vi "Burst Clock (Host).vi"() -> ()   [LabVIEW 2021]
uses:
  <vilib>/userDefined/High Color/nirio_resource_hc.ctl
  5a54fa91-9ec7-467a-a88a-b72ee3603559.vi
  <vilib>/rvi/interface/RandomDataEmulation/nirviRandomDataOpen.vi
  <vilib>/rvi/interface/common/niFpgaCacheSessionInfoDynamic.vi
  <vilib>/FPGAPlugInAG/Dynamic/niLvFpga_Run_Dynamic.vi
  <vilib>/Utility/error.llb/Error Cluster From Error Code.vi
  <vilib>/rvi/errors/niLvFpgaAdjustHostInterfaceError.vi
  <vilib>/FPGAPlugInAG/Dynamic/niLvFpga_Close_Dynamic.vi
  <vilib>/rvi/interface/nirviOpenFPGA/nirviOpenFPGA.xnode
  Burst Clock (FPGA).vi
  <vilib>/rvi/interface/nirviMethod/nirviMethod.xnode
  <vilib>/rvi/interface/nirviReadWriteControl/nirviReadWriteControl.xnode
  <vilib>/rvi/interface/nirviCloseFPGA/nirviCloseFPGA.xnode
  <vilib>/rvi/interface/Simulation/niFpgaSimulationCallBeginRW.vi
  <vilib>/FPGAPlugInAG/Dynamic/niLvFpga_Reset_Dynamic.vi
  NiFpgaLv.dll
  <vilib>/FPGAPlugInAG/Dynamic/niLvFpga_WriteFifo_Dynamic.vi
  <vilib>/rvi/errors/niLvFpgaMergeErrorWithErrorCode.vi
panel:
  in  "Resource Name":T1 caption="RIO Device"
  in  "Stop":bool
  in  "Go":bool
  in  "Array":cluster{"Clocks":u16, "Idle":u16}[](array[cluster])=[{"Clocks"=5, "Idle"=3}]
  out "error out":errorcluster
  in  "error in (no error)":errorcluster
  # "To Simulate:\n1. Navigate to \"Project -> Properties -> Conditional Disable Signals\" and set \"FPGA_SIM\" to \"TRUE\".\n2. Right-click on the FPGA Target and set \"Select Execution Mode\" to \"Simulation (Simulated I/O)\" \n\nTo Run on FPGA:\n1. Navigate to \"Project -> Properties -> Conditional Disable Signals\" and set \"FPGA_SIM\" to \"FALSE\".\n2. Right-click on the FPGA Target and set \"Select Execution Mode\" to \"FPGA Target\""
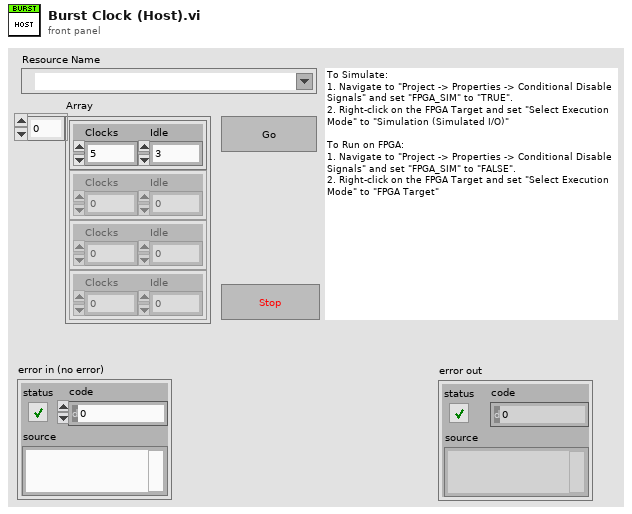
[diagram p1: front panel]
types:
  T1 = typedef "nirio_resource_hc.ctl" = tag
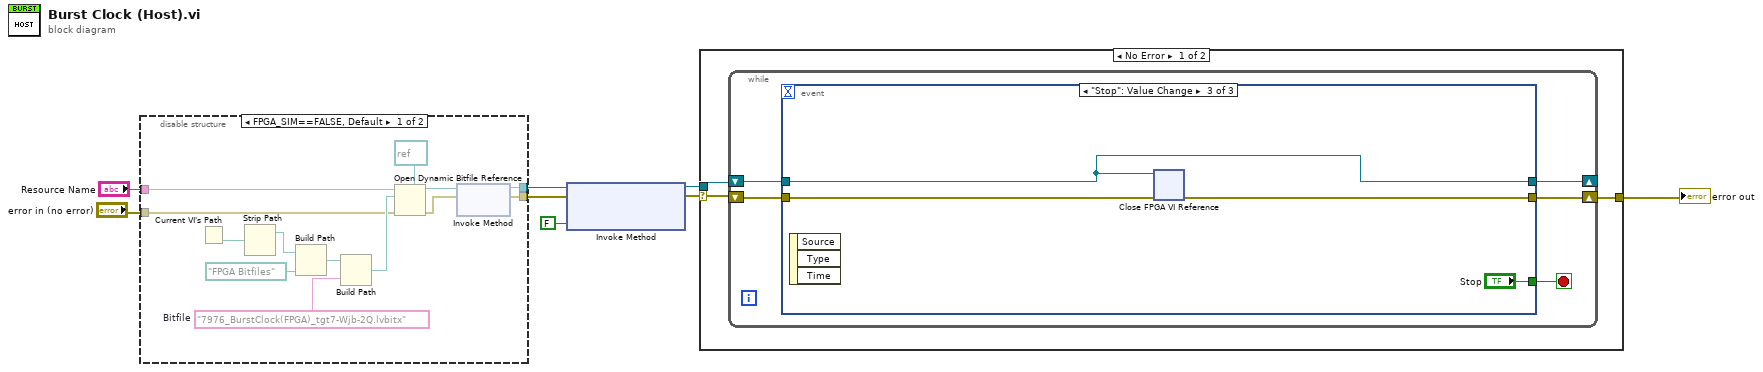
[diagram p0: block diagram]
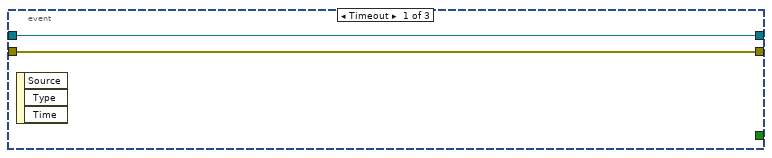
[diagram p2: hidden frame]
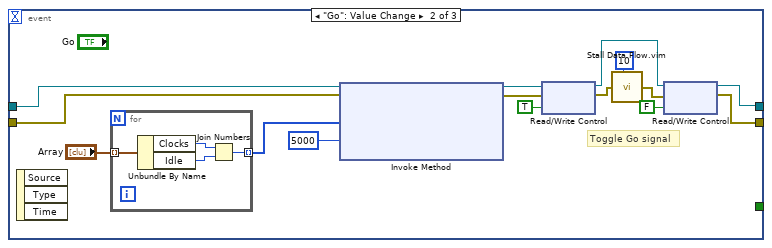
[diagram p3: hidden frame]
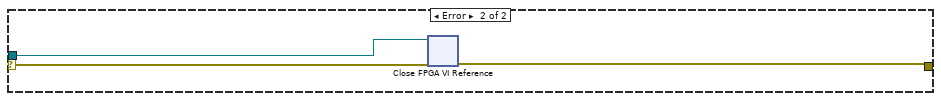
[diagram p4: hidden frame]
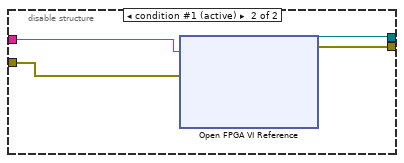
[diagram p5: hidden frame]
diagram:
  n1 = disable-structure shown="FPGA_SIM==FALSE, Default" {
    disable-tunnel: [w21 w23] -> w3
    disable-tunnel: [w20 w24] -> w4
    disable-tunnel: "error in (no error)" -> [w12 w25]
    disable-tunnel: "Resource Name" -> [w9 w22]
    frame condition #0 {
      w10 = "7976_BurstClock(FPGA)_tgt7-Wjb-2Q.lvbitx"  # Bitfile
      n2 = Current VI's Path() -> (path=w14:path)
      n3 = Strip Path(path=w14) -> (stripped path=w13:path)  [unwired: 1 out]
      n4 = Build Path(base path=w13, name or relative path=path "FPGA Bitfiles") -> (appended path=w18:path)
      n5 = Build Path(base path=w18, name or relative path=w10) -> (appended path=w19:path)
      n6 = Open Dynamic Bitfile Reference(0:w9, 1:w19, 3:w12, 4:refnum<k20> refnum ("FPGA Interface")) -> (5:w16:refnum<k20>, 8:w15:errorcluster)  [unwired: 1 in]
      n7 = xnode "Invoke Method"("FPGA VI Reference In"=w16, "error in"=w15) -> ("FPGA VI Reference Out"=w21:refnum<k20>, "error out"=w20:errorcluster)
    }
    frame condition #1 (active) {
      n8 = xnode "Open FPGA VI Reference"("error in"=w25, "resource name"=w22) -> ("FPGA VI Reference Out"=w23:refnum<k20>, "error out"=w24:errorcluster)
    }
  }
  n9 = xnode "Invoke Method"("FPGA VI Reference In"=w3, "error in"=w4, "Wait Until Done (F)"=FALSE) -> ("FPGA VI Reference Out"=w2:refnum<k20>, "error out"=w1:errorcluster)
  n10 = case shown="No Error" w1 {
    selector: w1 -> [w26 w61]
    tunnel: [w28 w59] -> w8
    tunnel: w2 -> [w27 w60]
    frame No Error {
      n11 = while {
        shift-right: [w30] -> w28
        shift-left: w26 -> [w33]
        shift-right: [w31] -> _
        shift-left: w27 -> [w32]
        stop <- w29 stop-if-true
        n12 = event shown="[2] \"Stop\": Value Change" {
          selector: _ -> [_ _ _]
          dyn-events: _ -> [_ _ _]
          timeout: _ -> [_ _ _]
          tunnel: w33 -> [w34 w50 w57]
          tunnel: w32 -> [w35 w49 w55]
          tunnel: [w35 w37 w55] -> w31
          tunnel: [w34 w38 w56] -> w30
          tunnel: [_ _ "Stop"] -> w29
          event Timeout {
            n13 = event-data() -> ()  [unwired: 1 in, 3 out]
          }
          event "Go": Value Change {
            # "Toggle Go signal"
            n14 = event-data() -> ()  [unwired: 1 in, 3 out]
            n15 = for {
              tunnel: "Array" -> [w54] mode=indexing
              tunnel: [w51] -> w47 mode=indexing
              n16 = Unbundle By Name(w54) -> ("Clocks"=w53:u16, "Idle"=w52:u16)
              n17 = Join Numbers(hi=w53, lo=w52) -> ((hi.lo)=w51:u32)
            }
            n18 = xnode "Invoke Method"("FPGA VI Reference In"=w49, "error in"=w50, "Data"=w47, "Timeout (ms)"=5000) -> ("FPGA VI Reference Out"=w45:refnum<k20>, "error out"=w44:errorcluster)  [unwired: 1 out]
            n19 = xnode "Read/Write Control"("FPGA VI Reference In"=w45, "error in"=w44, "Go"=TRUE) -> ("FPGA VI Reference Out"=w36:refnum<k20>, "error out"=w41:errorcluster)
            n20 = call "Stall Data Flow.vim"("value in"=w41, "milliseconds to wait"=u32 10) -> ("value out"=w40:errorcluster)  [unwired: 1 out]
            n21 = xnode "Read/Write Control"("FPGA VI Reference In"=w36, "error in"=w40, "Go"=FALSE) -> ("FPGA VI Reference Out"=w37:refnum<k20>, "error out"=w38:errorcluster)
          }
          event "Stop": Value Change {
            n22 = event-data() -> ()  [unwired: 1 in, 3 out]
            n23 = xnode "Close FPGA VI Reference"("FPGA VI Reference In"=w55, "error in"=w57) -> ("error out"=w56:errorcluster)
          }
        }
      }
    }
    frame Error {
      n24 = xnode "Close FPGA VI Reference"("FPGA VI Reference In"=w60, "error in"=w61) -> ("error out"=w59:errorcluster)
    }
  }
  "error out" <- w8
